vi "Initialize MeasurementLink Session.vi"(7 "remote connection options":T2, 8 "error in":errorcluster, 9 "initialize and close session behavior":T1, 10 "session initialization parameters":T3, 11 "session factory in":refnum<class "Session Factory.lvclass">) -> (0 "error out":errorcluster, 2 "session out":variant, 3 "session factory out":refnum<class "Session Factory.lvclass">)   [LabVIEW 2021, in "NI Session Management VISA.lvlib" / "Session Factory.lvclass"]
uses:
  Session Factory.lvclass
  Instrument/ISession Factory/Session Initialization Parameters.ctl
  Instrument/ISession Factory/Remote Connection Options.ctl
  Instrument/ISession Factory/Initialize and Close Session Behavior.ctl
  Session Factory.lvclass/Session Factory.ctl
  Instrument/ISession Factory/ISession Factory.lvclass
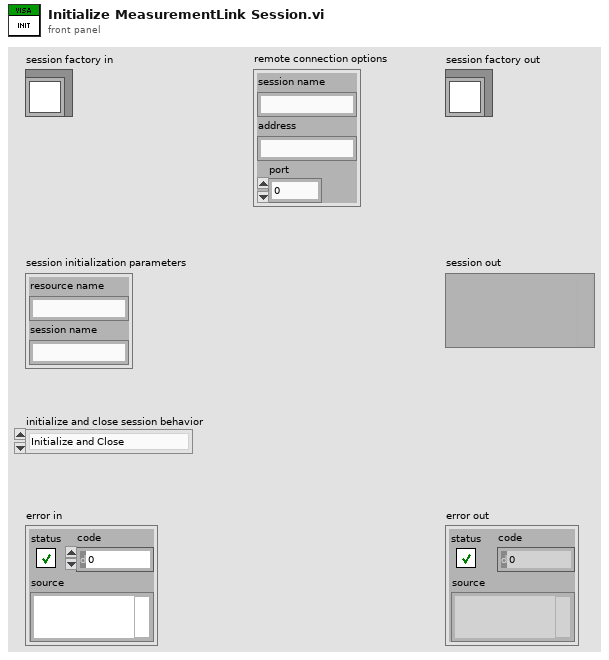
[diagram p1: front panel]
types:
  T1 = typedef "NI Session Management Instrument.lvlib/ISession Factory.lvclass/Initialize and Close Session Behavior.ctl" = enum16{"Initialize and Close", "Attach and Detach", "Initialize and Detach", "Attach and Close"}
  T2 = typedef "NI Session Management Instrument.lvlib/ISession Factory.lvclass/Remote Connection Options.ctl" = cluster{"session name":string, "address":string, "port":u32}
  T3 = typedef "NI Session Management Instrument.lvlib/ISession Factory.lvclass/Session Initialization Parameters.ctl" = cluster{"resource name":string, "session name":string}
  T4 = typedef "VISA Open Access Mode.ctl" = u32
  T5 = typedef "VISA gRPC Open Close Behavior.ctl" = enum16{"Auto", "Initialize and Close", "Attach and Detach", "Initialize and Detach", "Attach and Close"}
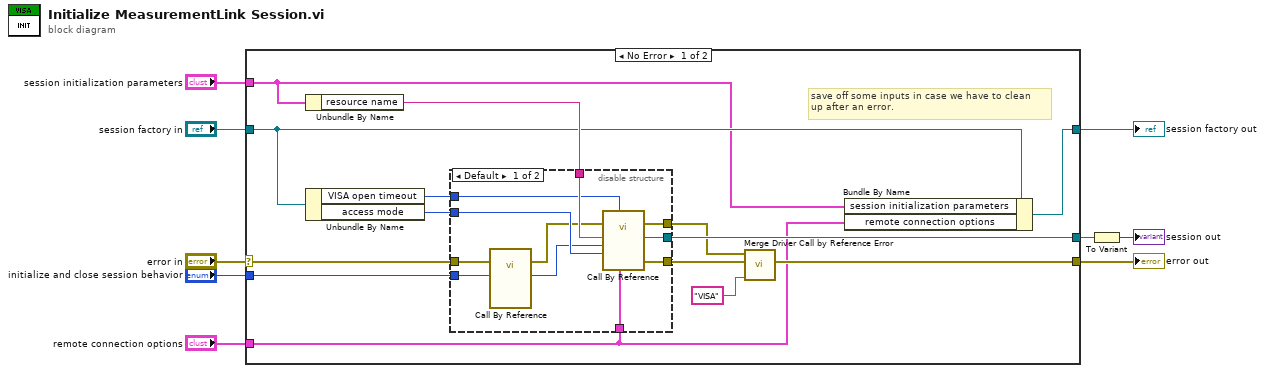
[diagram p0: block diagram]
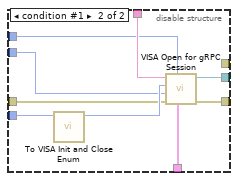
[diagram p2: hidden frame]
diagram:
  n1 = case shown="No Error" "error in" {
    selector: "error in" -> [w14 w44]
    tunnel: [w19 w44] -> w8
    tunnel: "session factory in" -> [w13 w45]
    tunnel: [w12 w45] -> w6
    tunnel: "remote connection options" -> [w11 _]
    tunnel: "session initialization parameters" -> [w10 _]
    tunnel: [w23 _] -> w3
    tunnel: "initialize and close session behavior" -> [w15 _]
    frame No Error {
      # "save off some inputs in case we have to clean\nup after an error."
      n2 = Unbundle By Name(w10) -> ("resource name"=w22:string)
      n3 = Unbundle By Name(w13) -> ("VISA open timeout"=w16:u32, "access mode"=w17:T4)
      n4 = disable-structure shown="Default" {
        disable-tunnel: [w34 w41] -> w23
        disable-tunnel: w22 -> [w33 w40]
        disable-tunnel: [w32 w43] -> w21
        disable-tunnel: [w31 _] -> w20
        disable-tunnel: w17 -> [w30 w37]
        disable-tunnel: w16 -> [w29 w36]
        disable-tunnel: w15 -> [w28 w39]
        disable-tunnel: w14 -> [w26 w35]
        disable-tunnel: w11 -> [w24 w42]
        frame condition #0 (active) {
          n5 = call-by-ref "?"(error in=w26, "factory init and close behavior"=w28) -> (error out=w25:errorcluster, "visa init and close behavior"=w27:T5)  [unwired: 11 in, 1 out]
          n6 = call-by-ref "?"(error in=w25, "gRPC Options"=w24, "VISA Open Timeout (0)"=w29, "Access Mode"=w30, "Open/Close Behavior"=w27, "VISA resource name"=w33) -> (error out=w31:errorcluster, 0:"error out"=w32:errorcluster, "VISA resource name out"=w34:refnum<visa-resource-name>)  [unwired: 6 in, 1 out]
        }
        frame condition #1 {
          n7 = call "To VISA Init and Close Enum.vi"("factory init and close behavior"=w39) -> ("visa init and close behavior"=w38:T5)  [unwired: 10 in]
          n8 = call <vilib>:"VISA Open for gRPC Session.vi"("gRPC Options"=w42, "VISA Open timeout (0)"=w36, "error in (no error)"=w35, "access mode (VISA Defaults)"=w37, "open/close behavior"=w38, "VISA resource name"=w40) -> ("error out"=w43:errorcluster, "VISA resource name out"=w41:refnum<visa-resource-name>)  [unwired: 4 in]
        }
      }
      n9 = call "Merge Driver Call by Reference Error.vi"("driver name"="VISA", "called vi error"=w21, "call by ref error"=w20) -> ("error out"=w19:errorcluster)  [unwired: 8 in]
      n10 = Bundle By Name(cluster=w13, "session initialization parameters"=w10, "remote connection options"=w11) -> (w12:refnum<class "Session Factory.lvclass">)
    }
    frame Error {
    }
  }
  "error out" <- w8
  "session factory out" <- w6
  n11 = To Variant(anything=w3) -> (Variant=→"session out":variant)
